vi "Launch Simulated IO.vi"(10 "Sim":bool, 11 "Bus Access":refnum<class "Local Bus.lvclass">[](array[class])) -> ()   [LabVIEW 2021]
uses:
  <vilib>/TSA/Omni-Bus/Local Bus/Local Bus.lvclass
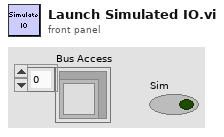
[diagram p1: front panel]
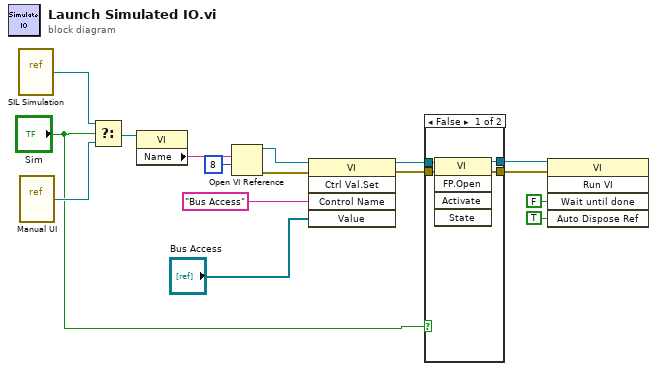
[diagram p0: block diagram]
diagram:
  n1 = vi-ref "SIL Simulation.vi"() -> (w4:refnum<vi>)
  n2 = vi-ref "Manual UI.vi"() -> (w2:refnum<vi>)
  n3 = Select(t=w4, s="Sim", f=w2) -> (s? t:f=w3:refnum<vi>)
  n4 = property class="VI"(reference=w3) -> ("Name"=w5:string)  [unwired: 1 in, 2 out]
  n5 = Open VI Reference(vi path=w5, options=8) -> (vi reference=w6:refnum<vi>, error out=w7:errorcluster)  [unwired: 4 in]
  n6 = invoke class="VI" method="Ctrl Val.Set"(reference=w6, error in=w7, "Control Name"="Bus Access", "Value"="Bus Access") -> (reference out=w13:refnum<vi>, error out=w14:errorcluster)  [unwired: 1 in, 3 out]
  n7 = case shown="False" "Sim" {
    tunnel: [w20 w21] -> w16
    tunnel: [w19 w22] -> w15
    tunnel: w14 -> [w18 w21]
    tunnel: w13 -> [w17 w22]
    frame False {
      n8 = invoke class="VI" method="FP.Open"(reference=w17, error in=w18) -> (reference out=w19:refnum<vi>, error out=w20:errorcluster)  [unwired: 3 in, 3 out]
    }
    frame True {
    }
  }
  n9 = invoke class="VI" method="Run VI"(reference=w15, error in=w16, "Wait until done"=FALSE ("Wait Until Done"), "Auto Dispose Ref"=TRUE ("Auto Dispose Reference")) -> ()  [unwired: 1 in, 5 out]
